vi "Get Connection Mode.vi"(8 "error in (no error)":errorcluster caption="错误输入（无错误）", 10 "nConnectedType":i32, 11 "nDevId":i32) -> (0 "error out":errorcluster caption="错误输出", 2 "nConnectedType out":i32, 3 "function return":i32)   [LabVIEW 2017, in "smncsftmt.lvlib"]
doc: "__declspec(dllexport) int GetConnectionMode(int nDevId, int* nConnectedType);"
uses:
  smncsftmt.lvlib
  smncsftmt.dll
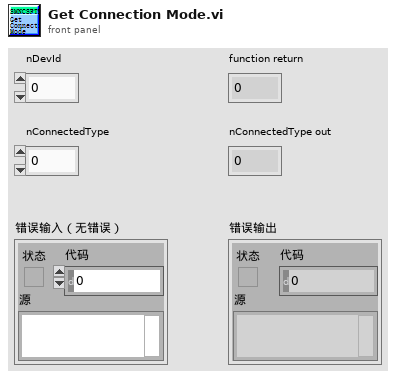
[diagram p1: front panel]
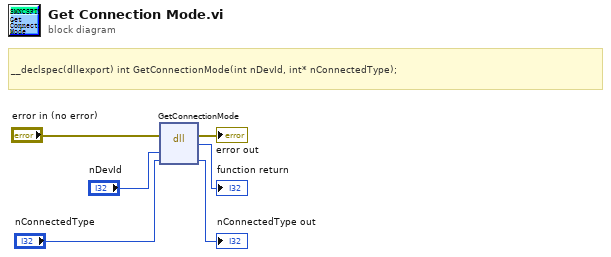
[diagram p0: block diagram]
diagram:
  # "__declspec(dllexport) int GetConnectionMode(int nDevId, int* nConnectedType);"
  n1 = dll-call lib="PTH2oabs CUsersaDesktop\nLABVIEW范例National InstrumentsLabVIEW 2017user.lib\tsmncsftmtsmncsftmt.*" fn="GetConnectionMode"(error in="error in (no error)", "nDevId"="nDevId", "nConnectedType"="nConnectedType") -> (error out=→"error out":errorcluster, →"function return":i32, "nConnectedType"=→"nConnectedType out":i32)  [unwired: 3 in, 1 out]
